vi "ReversedEngineering GetCaseStringConstants.vi"(0 "Diagram":refnum<vi>, 5 "error in (no error)":errorcluster) -> (15 "StringConstants":string[](array[string]), 16 "EventStructureUsed":bool, 19 "error out":errorcluster)   [LabVIEW 2020]
uses:
  <resource>/Framework/Providers/Open_GDS/UML/ReversedEngineering/ReversedEngineering QueuedStateMachinMemoryAction.ctl
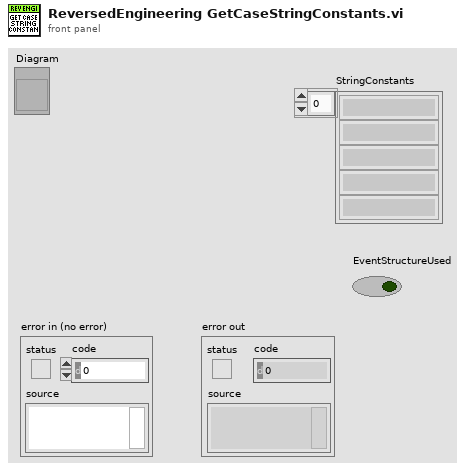
[diagram p1: front panel]
types:
  T1 = typedef "ReversedEngineering QueuedStateMachinMemoryAction.ctl" = enum16{"Initialize", "GetInsertQueuedArrayElementsVI", "SetQueuedStateJumps", "GetQueuedStateJumps"}
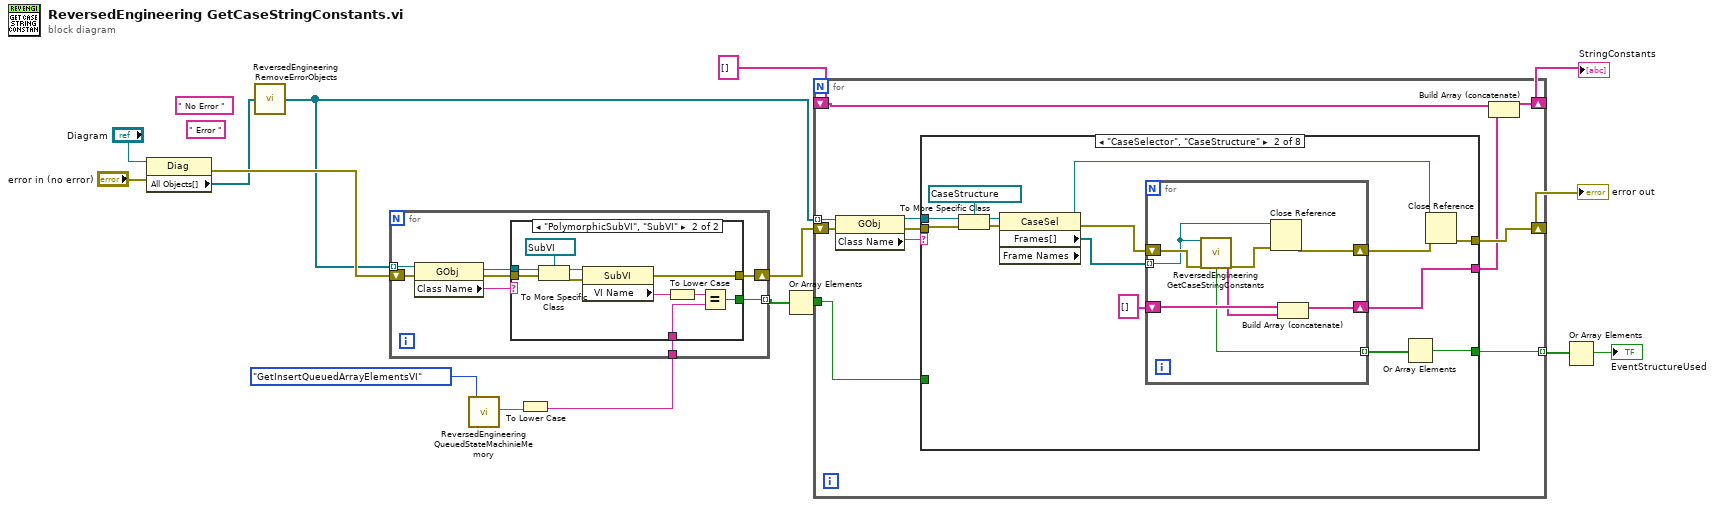
[diagram p0: block diagram]
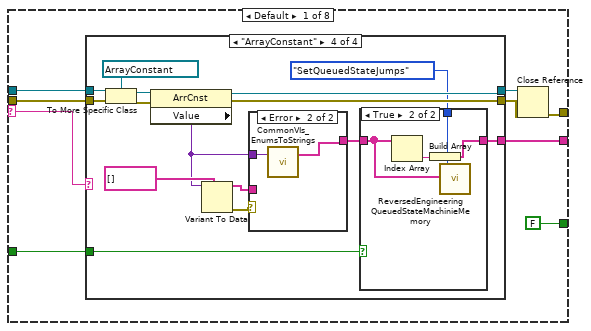
[diagram p3: hidden frame]
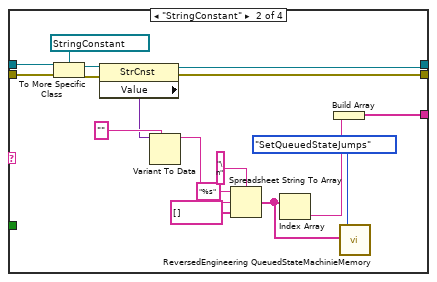
[diagram p5: hidden frame]
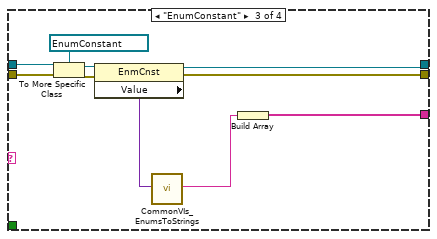
[diagram p6: hidden frame]
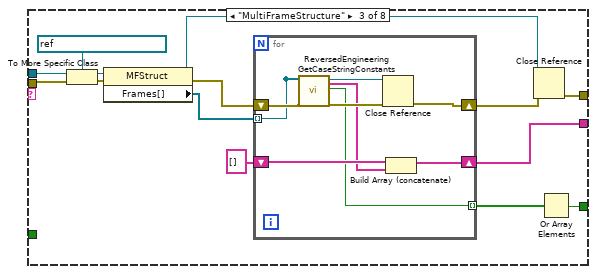
[diagram p9: hidden frame]
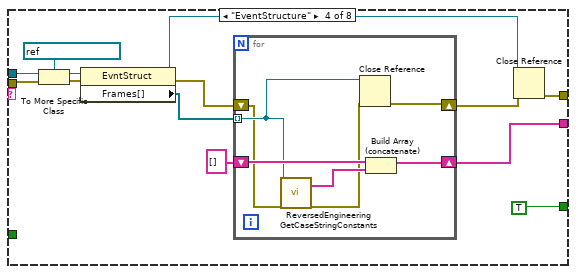
[diagram p10: hidden frame]
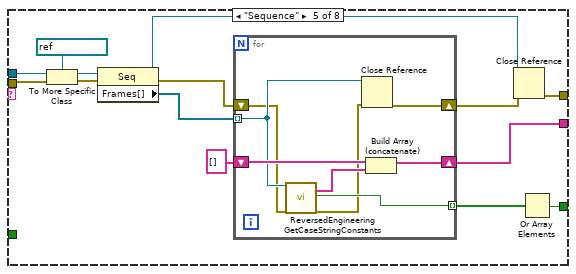
[diagram p11: hidden frame]
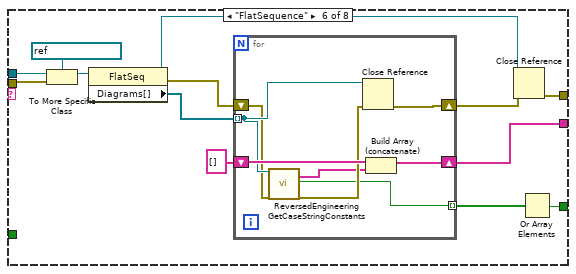
[diagram p12: hidden frame]
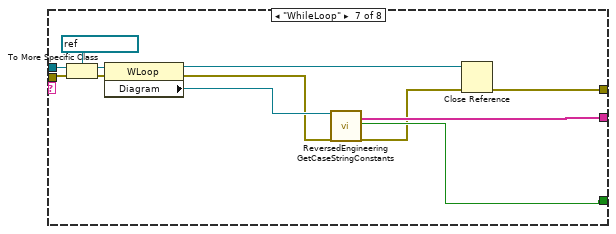
[diagram p13: hidden frame]
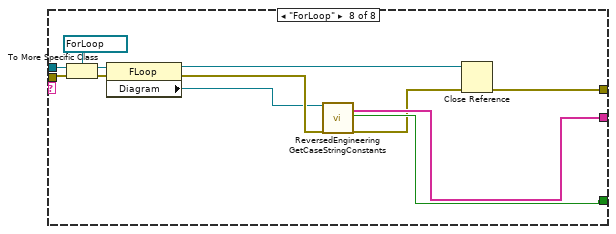
[diagram p14: hidden frame]
diagram:
  (unwired) " Error "
  (unwired) " No Error "
  n1 = property class="Diag"(reference="Diagram", error in="error in (no error)") -> (error out=w6:errorcluster, "All Objects[]"=w2:refnum<vi>[])  [unwired: 1 out]
  n2 = call <resource>:"ReversedEngineering RemoveErrorObjects.vi"("ObjectsIn"=w2) -> ("ObjectsOut"=w1:refnum<vi>[])
  n3 = call <resource>:"ReversedEngineering QueuedStateMachinieMemory.vi"("Action(GetInsertQueuedArrayElementsVI)"=ReversedEngineering_QueuedStateMachinMemoryAction."GetInsertQueuedArrayElementsVI" ("Action(GetInsertQueuedArrayElements)")) -> ("VIName"=w8:string)  [unwired: 3 in, 15 out]
  n4 = To Lower Case(string=w8) -> (all lower case string=w7:string)
  n5 = for {
    tunnel: w1 -> [w24] mode=indexing
    shift-right: [w17] -> w5
    shift-left: w6 -> [w22]
    tunnel: w7 -> [w19]
    tunnel: [w18] -> w4 mode=indexing
    n6 = property class="GObj"(reference=w24, error in=w22) -> (reference out=w21:refnum<vi>, error out=w20:errorcluster, "Class Name"=w23:string)
    n7 = case shown="\"PolymorphicSubVI\", \"SubVI\"" w23 {
      tunnel: w21 -> [_ w35]
      tunnel: w20 -> [w25 w33]
      tunnel: w19 -> [_ w29]
      tunnel: [_ w28] -> w18
      tunnel: [w25 w27] -> w17
      frame "False", Default {
      }
      frame "PolymorphicSubVI", "SubVI" {
        n8 = To More Specific Class(target class=refnum<vi> refnum ("WhileLoop"), reference=w35, error in=w33) -> (specific class reference=w32:refnum<vi>, error out=w26:errorcluster)
        n9 = property class="SubVI"(reference=w32, error in=w26) -> (error out=w27:errorcluster, "VI Name"=w31:string)  [unwired: 1 out]
        n10 = To Lower Case(string=w31) -> (all lower case string=w30:string)
        n11 = Equal?(x=w30, y=w29) -> (x = y?=w28:bool)
      }
    }
  }
  n12 = Or Array Elements(Boolean array=w4) -> (logical OR=w3:bool)
  n13 = for {
    tunnel: w1 -> [w46] mode=indexing
    shift-right: [w41] -> w14
    shift-left: w5 -> [w43]
    shift-right: [w39] -> w13
    shift-left: string[] [] -> [w40]
    tunnel: [w37] -> w11 mode=indexing
    tunnel: w3 -> [w36]
    n14 = property class="GObj"(reference=w46, error in=w43) -> (reference out=w44:refnum<vi>, error out=w42:errorcluster, "Class Name"=w45:string)
    n15 = case shown="\"CaseSelector\", \"CaseStructure\"" w45 {
      selector: w45 -> [w54 _ _ _ _ _ _ _]
      tunnel: w44 -> [w52 w121 w143 w164 w185 w206 w226 w238]
      tunnel: w42 -> [w53 w116 w139 w161 w181 w205 w221 w233]
      tunnel: [w55 w115 w138 w160 w180 w204 w215 w227] -> w41
      tunnel: [w49 w112 w135 w157 w178 w202 w218 w230] -> w38
      tunnel: [FALSE ("EventStructureUsed") w109 w132 TRUE w174 w196 w217 w229] -> w37
      tunnel: w36 -> [w47 _ _ _ _ _ _ _]
      frame Default {
        n16 = case shown="\"ArrayConstant\"" w54 {
          tunnel: w53 -> [w57 w72 w82 w97]
          tunnel: w52 -> [w56 w73 w83 w98]
          tunnel: [w57 w69 w79 w95] -> w51
          tunnel: [w56 w68 w78 w94] -> w50
          tunnel: [_ w70 w80 w86] -> w49
          tunnel: w47 -> [_ _ _ w88]
          frame "False", Default {
          }
          frame "StringConstant" {
            n17 = To More Specific Class(target class=refnum<vi> refnum ("WhileLoop"), reference=w73, error in=w72) -> (specific class reference=w71:refnum<vi>, error out=w67:errorcluster)
            n18 = property class="StrCnst"(reference=w71, error in=w67) -> (reference out=w68:refnum<vi>, error out=w69:errorcluster, "Value"=w65:variant)
            n19 = Variant To Data(type="", Variant=w65) -> (data=w61:string)  [unwired: 1 in, 1 out]
            n20 = Spreadsheet String To Array(delimiter (Tab)="\n", format string="%s", spreadsheet string=w61, array type (2D Dbl)=string[] []) -> (array=w59:string[])
            n21 = Index Array(array=w59) -> (element=w60:string)  [unwired: 1 in]
            n22 = Build Array(w60) -> (w70:string[])
            n23 = call <resource>:"ReversedEngineering QueuedStateMachinieMemory.vi"("StateJumps"=w59, "Action(GetInsertQueuedArrayElementsVI)"=ReversedEngineering_QueuedStateMachinMemoryAction."SetQueuedStateJumps") -> ()  [unwired: 2 in, 16 out]
          }
          frame "EnumConstant" {
            n24 = To More Specific Class(target class=refnum<vi> refnum ("WhileLoop"), reference=w83, error in=w82) -> (specific class reference=w81:refnum<vi>, error out=w77:errorcluster)
            n25 = property class="EnmCnst"(reference=w81, error in=w77) -> (reference out=w78:refnum<vi>, error out=w79:errorcluster, "Value"=w76:variant)
            n26 = call <resource>:"CommonVIs_EnumsToStrings.vi"("SingleEnumVariantIn"=w76) -> ("EnumItem"=w75:string)  [unwired: 2 in, 16 out]
            n27 = Build Array(w75) -> (w80:string[])
          }
          frame "ArrayConstant" {
            n28 = To More Specific Class(target class=refnum<vi> refnum ("WhileLoop"), reference=w98, error in=w97) -> (specific class reference=w96:refnum<vi>, error out=w93:errorcluster)
            n29 = property class="ArrCnst"(reference=w96, error in=w93) -> (reference out=w94:refnum<vi>, error out=w95:errorcluster, "Value"=w90:variant)
            n30 = Variant To Data(type=string[] [], Variant=w90) -> (data=w89:string[], error out=w91:errorcluster)  [unwired: 1 in]
            n31 = case shown="Error" w91 {
              tunnel: w90 -> [_ w107]
              tunnel: w89 -> [w105 _]
              tunnel: [w105 w106] -> w87
              frame No Error {
              }
              frame Error {
                n32 = call <resource>:"CommonVIs_EnumsToStrings.vi"("ArrayEnumVariantIn"=w107) -> ("EnumItems(string)"=w106:string[])  [unwired: 2 in, 16 out]
              }
            }
            n33 = case shown="True" w88 {
              tunnel: w87 -> [w100 w102]
              tunnel: [w100 w103] -> w86
              tunnel: ReversedEngineering_QueuedStateMachinMemoryAction."SetQueuedStateJumps" ("Action(GetInsertQueuedArrayElementsVI)") -> [_ w104]
              frame False {
              }
              frame True {
                n34 = Index Array(array=w102) -> (element=w101:string)  [unwired: 1 in]
                n35 = Build Array(w101) -> (w103:string[])
                n36 = call <resource>:"ReversedEngineering QueuedStateMachinieMemory.vi"("StateJumps"=w102, "Action(GetInsertQueuedArrayElementsVI)"=w104) -> ()  [unwired: 2 in, 16 out]
              }
            }
          }
        }
        n37 = Close Reference(reference=w50, error in (no error)=w51) -> (error out=w55:errorcluster)
      }
      frame "CaseSelector", "CaseStructure" {
        n38 = To More Specific Class(target class=refnum<vi> refnum ("CaseSelector"), reference=w121, error in=w116) -> (specific class reference=w119:refnum<vi>, error out=w117:errorcluster)
        n39 = property class="CaseSel" props=["Frames[]", "Frame Names"](reference=w119, error in=w117) -> (reference out=w114:refnum<vi>, error out=w108:errorcluster, "Frames[]"=w118:refnum<vi>[])  [unwired: 1 out]
        n40 = for {
          tunnel: w118 -> [w122] mode=indexing
          shift-right: [w127] -> w113
          shift-left: w108 -> [w124]
          shift-right: [w128] -> w112
          shift-left: string[] [] -> [w129]
          tunnel: [w126] -> w110 mode=indexing
          n41 = call <resource>:"ReversedEngineering GetCaseStringConstants.vi"("Diagram"=w122, "error in (no error)"=w124) -> ("StringConstants"=w125:string[], "EventStructureUsed"=w126:bool, "error out"=w123:errorcluster)  [unwired: 15 in]
          n42 = Close Reference(reference=w122, error in (no error)=w123) -> (error out=w127:errorcluster)
          n43 = Build Array (concatenate)(w129, w125) -> (w128:string[])
        }
        n44 = Or Array Elements(Boolean array=w110) -> (logical OR=w109:bool)
        n45 = Close Reference(reference=w114, error in (no error)=w113) -> (error out=w115:errorcluster)
      }
      frame "MultiFrameStructure" {
        n46 = To More Specific Class(target class=refnum<vi> refnum ("MultiFrameStructure"), reference=w143, error in=w139) -> (specific class reference=w142:refnum<vi>, error out=w140:errorcluster)
        n47 = property class="MFStruct"(reference=w142, error in=w140) -> (reference out=w137:refnum<vi>, error out=w130:errorcluster, "Frames[]"=w141:refnum<vi>[])
        n48 = for {
          tunnel: w141 -> [w146] mode=indexing
          shift-right: [w149] -> w136
          shift-left: w130 -> [w148]
          shift-right: [w150] -> w135
          shift-left: string[] [] -> [w151]
          tunnel: [w144] -> w131 mode=indexing
          n49 = call <resource>:"ReversedEngineering GetCaseStringConstants.vi"("Diagram"=w146, "error in (no error)"=w148) -> ("StringConstants"=w145:string[], "EventStructureUsed"=w144:bool, "error out"=w147:errorcluster)  [unwired: 15 in]
          n50 = Close Reference(reference=w146, error in (no error)=w147) -> (error out=w149:errorcluster)
          n51 = Build Array (concatenate)(w151, w145) -> (w150:string[])
        }
        n52 = Close Reference(reference=w137, error in (no error)=w136) -> (error out=w138:errorcluster)
        n53 = Or Array Elements(Boolean array=w131) -> (logical OR=w132:bool)
      }
      frame "EventStructure" {
        n54 = To More Specific Class(target class=refnum<vi> refnum ("EventStructure"), reference=w164, error in=w161) -> (specific class reference=w154:refnum<vi>, error out=w162:errorcluster)
        n55 = property class="EvntStruct"(reference=w154, error in=w162) -> (reference out=w159:refnum<vi>, error out=w152:errorcluster, "Frames[]"=w163:refnum<vi>[])
        n56 = for {
          tunnel: w163 -> [w167] mode=indexing
          shift-right: [w169] -> w158
          shift-left: w152 -> [w166]
          shift-right: [w170] -> w157
          shift-left: string[] [] -> [w171]
          n57 = call <resource>:"ReversedEngineering GetCaseStringConstants.vi"("Diagram"=w167, "error in (no error)"=w166) -> ("StringConstants"=w168:string[], "error out"=w165:errorcluster)  [unwired: 15 in, 1 out]
          n58 = Close Reference(reference=w167, error in (no error)=w165) -> (error out=w169:errorcluster)
          n59 = Build Array (concatenate)(w171, w168) -> (w170:string[])
        }
        n60 = Close Reference(reference=w159, error in (no error)=w158) -> (error out=w160:errorcluster)
      }
      frame "Sequence" {
        n61 = To More Specific Class(target class=refnum<vi> refnum ("Sequence"), reference=w185, error in=w181) -> (specific class reference=w184:refnum<vi>, error out=w182:errorcluster)
        n62 = property class="Seq"(reference=w184, error in=w182) -> (reference out=w179:refnum<vi>, error out=w172:errorcluster, "Frames[]"=w183:refnum<vi>[])
        n63 = for {
          tunnel: w183 -> [w188] mode=indexing
          shift-right: [w191] -> w175
          shift-left: w172 -> [w186]
          shift-right: [w192] -> w178
          shift-left: string[] [] -> [w193]
          tunnel: [w190] -> w173 mode=indexing
          n64 = call <resource>:"ReversedEngineering GetCaseStringConstants.vi"("Diagram"=w188, "error in (no error)"=w186) -> ("StringConstants"=w189:string[], "EventStructureUsed"=w190:bool, "error out"=w187:errorcluster)  [unwired: 15 in]
          n65 = Close Reference(reference=w188, error in (no error)=w187) -> (error out=w191:errorcluster)
          n66 = Build Array (concatenate)(w193, w189) -> (w192:string[])
        }
        n67 = Close Reference(reference=w179, error in (no error)=w175) -> (error out=w180:errorcluster)
        n68 = Or Array Elements(Boolean array=w173) -> (logical OR=w174:bool)
      }
      frame "FlatSequence" {
        n69 = To More Specific Class(target class=refnum<vi> refnum ("FlatSequence"), reference=w206, error in=w205) -> (specific class reference=w199:refnum<vi>)  [unwired: 1 out]
        n70 = property class="FlatSeq"(reference=w199) -> (reference out=w197:refnum<vi>, error out=w194:errorcluster, "Diagrams[]"=w198:refnum<vi>[])  [unwired: 1 in]
        n71 = for {
          tunnel: w198 -> [w211] mode=indexing
          shift-right: [w212] -> w203
          shift-left: w194 -> [w210]
          shift-right: [w213] -> w202
          shift-left: string[] [] -> [w214]
          tunnel: [w208] -> w195 mode=indexing
          n72 = call <resource>:"ReversedEngineering GetCaseStringConstants.vi"("Diagram"=w211, "error in (no error)"=w210) -> ("StringConstants"=w207:string[], "EventStructureUsed"=w208:bool, "error out"=w209:errorcluster)  [unwired: 15 in]
          n73 = Close Reference(reference=w211, error in (no error)=w209) -> (error out=w212:errorcluster)
          n74 = Build Array (concatenate)(w214, w207) -> (w213:string[])
        }
        n75 = Close Reference(reference=w197, error in (no error)=w203) -> (error out=w204:errorcluster)
        n76 = Or Array Elements(Boolean array=w195) -> (logical OR=w196:bool)
      }
      frame "WhileLoop" {
        n77 = To More Specific Class(target class=refnum<vi> refnum ("WhileLoop"), reference=w226, error in=w221) -> (specific class reference=w225:refnum<vi>, error out=w222:errorcluster)
        n78 = property class="WLoop"(reference=w225, error in=w222) -> (reference out=w223:refnum<vi>, error out=w219:errorcluster, "Diagram"=w220:refnum<vi>)
        n79 = call <resource>:"ReversedEngineering GetCaseStringConstants.vi"("Diagram"=w220, "error in (no error)"=w219) -> ("StringConstants"=w218:string[], "EventStructureUsed"=w217:bool, "error out"=w216:errorcluster)  [unwired: 15 in]
        n80 = Close Reference(reference=w223, error in (no error)=w216) -> (error out=w215:errorcluster)
      }
      frame "ForLoop" {
        n81 = To More Specific Class(target class=refnum<vi> refnum ("WhileLoop"), reference=w238, error in=w233) -> (specific class reference=w237:refnum<vi>, error out=w234:errorcluster)
        n82 = property class="FLoop"(reference=w237, error in=w234) -> (reference out=w235:refnum<vi>, error out=w232:errorcluster, "Diagram"=w231:refnum<vi>)
        n83 = call <resource>:"ReversedEngineering GetCaseStringConstants.vi"("Diagram"=w231, "error in (no error)"=w232) -> ("StringConstants"=w230:string[], "EventStructureUsed"=w229:bool, "error out"=w228:errorcluster)  [unwired: 15 in]
        n84 = Close Reference(reference=w235, error in (no error)=w228) -> (error out=w227:errorcluster)
      }
    }
    n85 = Build Array (concatenate)(w40, w38) -> (w39:string[])
  }
  "error out" <- w14
  "StringConstants" <- w13
  n86 = Or Array Elements(Boolean array=w11) -> (logical OR=→"EventStructureUsed":bool)
